vi "P9_AbortIdle.vi"(11 "Inputs":string[](array[string])) -> (2 "Output/Failure":string, 3 "CLI Process Return Code":i32)   [LabVIEW 2026]
doc: "Slice 1.1 probe: Control: Open VI Reference, Abort VI on a VI that is not running, read state, close the reference."
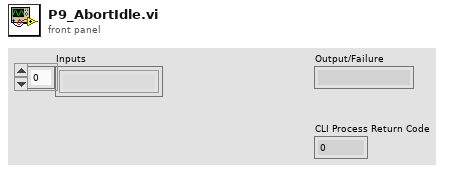
[diagram p1: front panel]
types:
  T1 = enum32{"Bad", "Idle", "Run top level", "Running"}
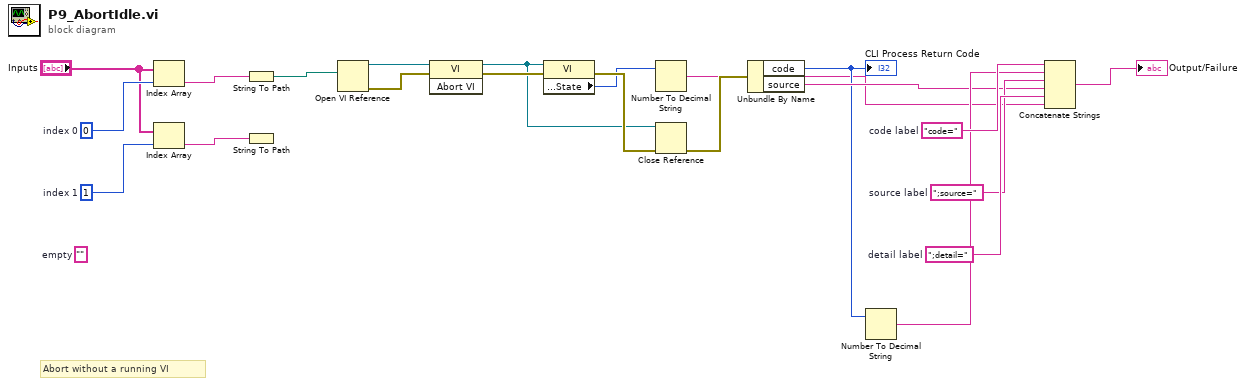
[diagram p0: block diagram]
diagram:
  w20 = ";detail="  # detail label
  w19 = ";source="  # source label
  w18 = "code="  # code label
  (unwired) ""  # empty
  w3 = 1  # index 1
  w2 = 0  # index 0
  # "Abort without a running VI"
  n1 = Index Array(array="Inputs", index=w2) -> (element=w4:string)
  n2 = Index Array(array="Inputs", index=w3) -> (element=w5:string)
  n3 = String To Path(string=w4) -> (path=w6:path)
  n4 = String To Path(string=w5) -> ()  [unwired: 1 out]
  n5 = Open VI Reference(vi path=w6) -> (vi reference=w7:refnum<vi>, error out=w8:errorcluster)  [unwired: 5 in]
  n6 = invoke class="VI" method="Abort VI"(reference=w7, error in=w8) -> (reference out=w9:refnum<vi>, error out=w10:errorcluster)  [unwired: 1 in, 1 out]
  n7 = property class="VI"(reference=w9, error in=w10) -> (error out=w12:errorcluster, "Execution:State"=w11:T1)  [unwired: 1 out]
  n8 = Number To Decimal String(number=w11) -> (decimal integer string=w13:string)  [unwired: 1 in]
  n9 = Close Reference(reference=w9, error in (no error)=w12) -> (error out=w14:errorcluster)
  n10 = Unbundle By Name(w14) -> ("code"=w15:i32, "source"=w16:string)
  "CLI Process Return Code" <- w15
  n11 = Number To Decimal String(number=w15) -> (decimal integer string=w17:string)  [unwired: 1 in]
  n12 = Concatenate Strings(w18, w17, w19, w16, w20, w13) -> (→"Output/Failure":string)
